vi "Registry_Stale_Scan.vi"(8 "error in (no error)":errorcluster={"status"=FALSE, "code"=0, "source"="\"\""}, 10 "freshness limits":string, 11 "Registry values":string) -> (0 "error out":errorcluster={"status"=FALSE, "code"=0, "source"="\"\""}, 2 "status ok":bool, 3 "Quality transition events":string)   [LabVIEW 2026]
doc: "INTENT: Mark expired feedback quality. LOGIC: Compare last update times and mark stale; publish equipment health events when configured."
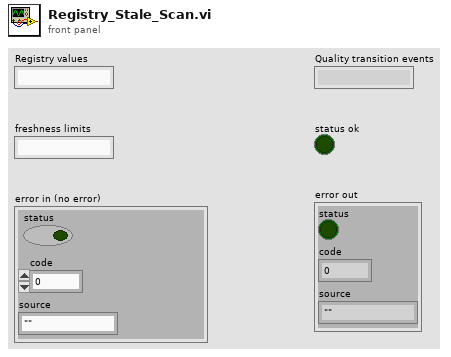
[diagram p1: front panel]
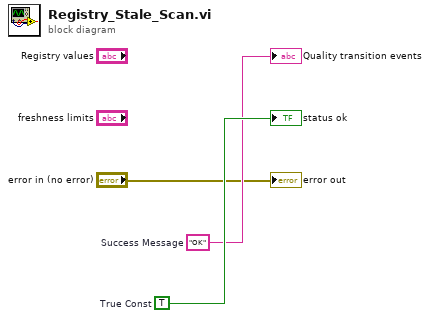
[diagram p0: block diagram]
diagram:
  w3 = TRUE  # True Const
  w2 = "OK"  # Success Message
  "Quality transition events" <- w2
  "status ok" <- w3
  "error out" <- "error in (no error)"
